vi "Update RH.vi"(8 "error in":errorcluster, 10 "Gas Humidity":dbl, 11 "DeepU Results in":refnum<class "DeepU Results.lvclass">) -> (0 "error out":errorcluster, 3 "DeepU Results out":refnum<class "DeepU Results.lvclass">)   [LabVIEW 2019, in "Results.lvlib" / "DeepU Results.lvclass"]
uses:
  DeepU Results.lvclass
  DeepU Results.lvclass/DeepU Results.ctl
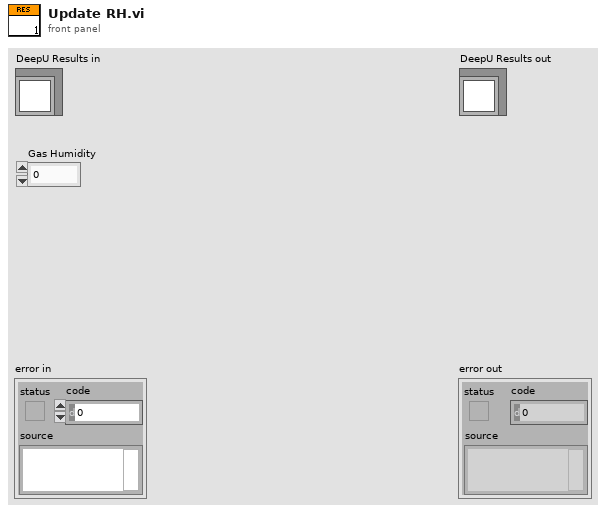
[diagram p1: front panel]
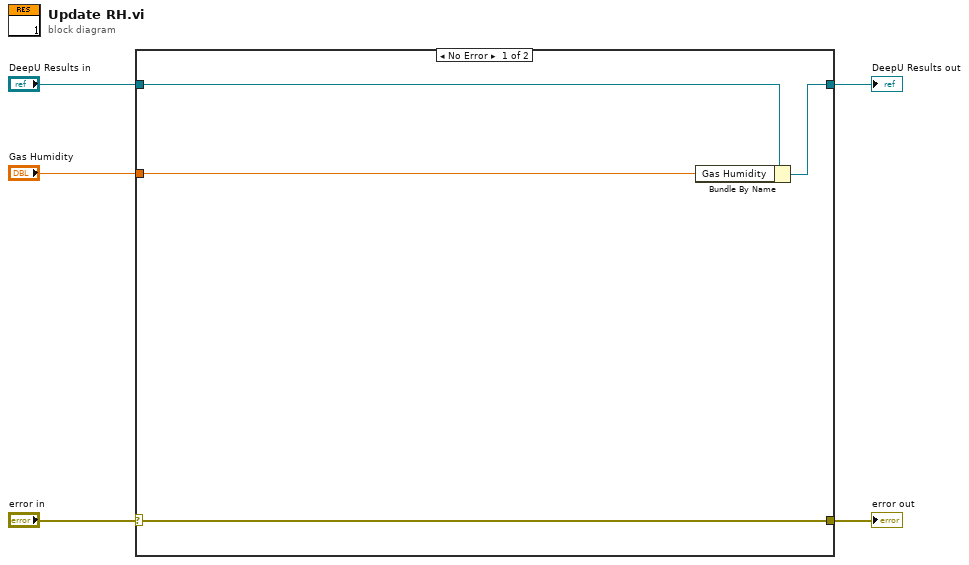
[diagram p0: block diagram]
diagram:
  n1 = case shown="No Error" "error in" {
    selector: "error in" -> [w9 w10]
    tunnel: [w9 w10] -> w2
    tunnel: [w8 w11] -> w3
    tunnel: "DeepU Results in" -> [w7 w11]
    tunnel: "Gas Humidity" -> [w6 _]
    frame No Error {
      n2 = Bundle By Name(cluster=w7, "Gas Humidity"=w6) -> (w8:refnum<class "DeepU Results.lvclass">)
    }
    frame Error {
    }
  }
  "error out" <- w2
  "DeepU Results out" <- w3
